vi "lvmcp_fire.vi"() -> ()   [LabVIEW 2015]
panel:
  out "error out":errorcluster
  in  "reference":refnum<vi>
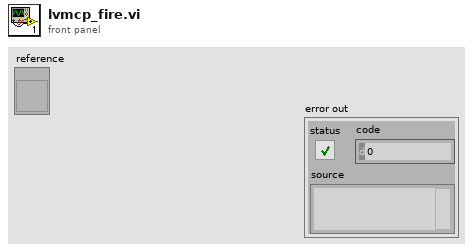
[diagram p1: front panel]
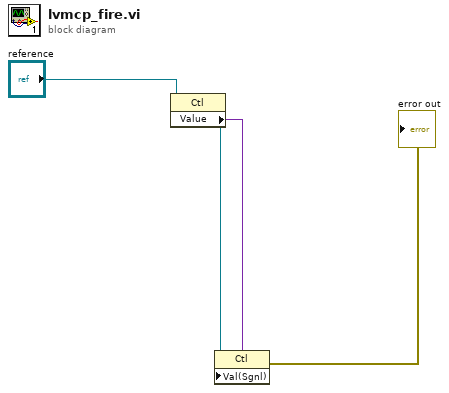
[diagram p0: block diagram]
diagram:
  n1 = property class="Ctl"(reference="reference") -> (reference out=w4:refnum<vi>, error out=w2:errorcluster, "Value"=w3:variant)  [unwired: 1 in]
  n2 = property class="Ctl"(reference=w4, error in=w2, "Val(Sgnl)"=w3) -> (error out=→"error out":errorcluster)  [unwired: 1 out]
